vi "ZM-CI-handlePackage.vi"(8 "error in (no error)":errorcluster, 10 "package":refnum<class "ZM-PC-package.lvclass">, 11 "ZM-ROOT-root in":refnum<class "ZM-ROOT-root.lvclass">) -> (0 "error out":errorcluster, 3 "ZM-ROOT-root out":refnum<class "ZM-ROOT-root.lvclass">)   [LabVIEW 2020, in "ZM-ROOT-root.lvlib" / "ZM-ROOT-root.lvclass"]
doc: "The root's ZM-CI-handlePackage override: routes every package by destination. Communication: noted and forwarded to the communication manager while it runs. Root: an error package is shown on the panel, any other is noted. Unknown and Hardware: dropped with one line in the error log (not an error)."
uses:
  ZM-ROOT-root.lvclass
  common/ZM-PC-packages/ZM-PC-package/ZM-PC-package.lvclass
  ZM-ROOT-root.lvclass/ZM-ROOT-root.ctl
  common/ZM-CI-common_interfaces/ZM-CI-handlePackage Msg/ZM-CI-handlePackage Msg.lvclass
  <vilib>/ActorFramework/Message Enqueuer/Message Enqueuer.lvclass
  common/ZM-CU-common_utilities/ZM-CU-common_utilities.lvlib
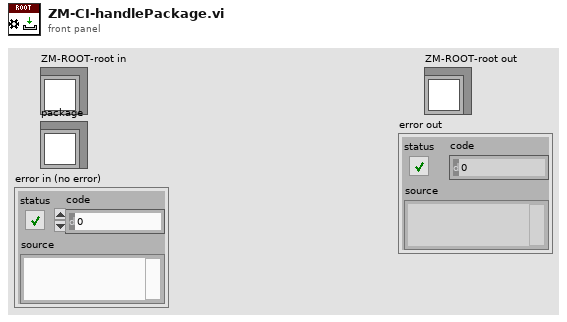
[diagram p1: front panel]
types:
  T1 = typedef "ZM-PC-packages.lvlib/ZM-PC-package.lvclass/ZM-PC-DESTINATION.ctl" = enum16{"Unknown", "Root", "Hardware", "Communication"}
  T2 = typedef "ZM-PC-packages.lvlib/ZM-PC-package.lvclass/ZM-PC-PACKAGE_TYPE.ctl" = enum16{"Undefined", "TestPackage", "ErrorPackage"}
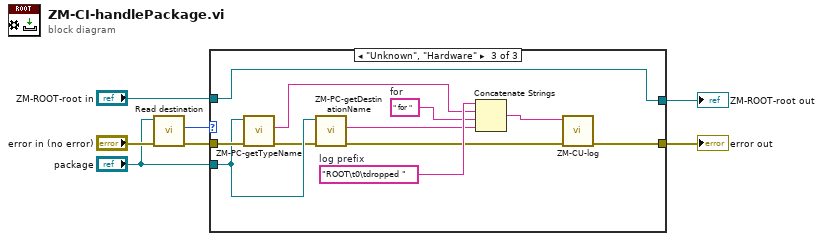
[diagram p0: block diagram]
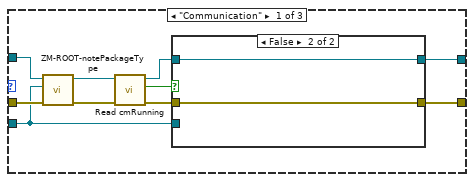
[diagram p2: hidden frame]
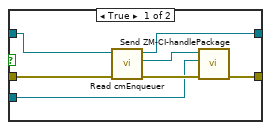
[diagram p3: hidden frame]
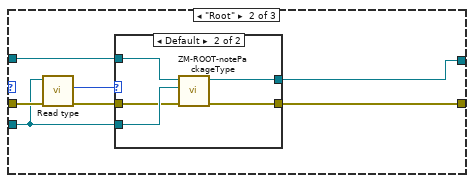
[diagram p4: hidden frame]
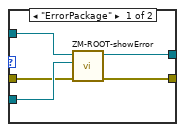
[diagram p5: hidden frame]
diagram:
  n1 = call "Read destination.vi"("error in (no error)"="error in (no error)", "ZM-PC-package in"="package") -> ("error out"=w4:errorcluster, "ZM-PC-DESTINATION"=w3:T1)  [unwired: 7 in, 1 out]
  n2 = case shown="\"Unknown\", \"Hardware\"" w3 {
    tunnel: "ZM-ROOT-root in" -> [w17 w32 w45]
    tunnel: "package" -> [w12 w31 w53]
    tunnel: w4 -> [w16 w33 w54]
    tunnel: [w9 w28 w45] -> w2
    tunnel: [w8 w27 w44] -> w1
    frame "Communication" {
      n3 = call "ZM-ROOT-notePackageType.vi"("error in (no error)"=w16, "package"=w12, "ZM-ROOT-root in"=w17) -> ("error out"=w15:errorcluster, "ZM-ROOT-root out"=w14:refnum<class "ZM-ROOT-root.lvclass">)  [unwired: 7 in]
      n4 = call "Read cmRunning.vi"("error in (no error)"=w15, "ZM-ROOT-root in"=w14) -> ("error out"=w11:errorcluster, "cmRunning"=w10:bool, "ZM-ROOT-root out"=w13:refnum<class "ZM-ROOT-root.lvclass">)  [unwired: 7 in]
      n5 = case shown="False" w10 {
        tunnel: w13 -> [w23 w26]
        tunnel: w12 -> [w20 _]
        tunnel: w11 -> [w24 w25]
        tunnel: [w19 w26] -> w9
        tunnel: [w18 w25] -> w8
        frame True {
          n6 = call "Read cmEnqueuer.vi"("error in (no error)"=w24, "ZM-ROOT-root in"=w23) -> ("error out"=w21:errorcluster, "Actor Framework:Message Enqueuer"=w22:refnum<class "Message Enqueuer.lvclass">, "ZM-ROOT-root out"=w19:refnum<class "ZM-ROOT-root.lvclass">)  [unwired: 7 in]
          n7 = call "Send ZM-CI-handlePackage.vi"("error in (no error)"=w21, "package"=w20, "Message Enqueuer"=w22) -> ("error out"=w18:errorcluster)  [unwired: 7 in, 1 out]
        }
        frame False {
        }
      }
    }
    frame "Root" {
      n8 = call "Read type.vi"("error in (no error)"=w33, "ZM-PC-package in"=w31) -> ("error out"=w30:errorcluster, "ZM-PC-PACKAGE_TYPE"=w29:T2)  [unwired: 7 in, 1 out]
      n9 = case shown="Default" w29 {
        tunnel: w32 -> [w38 w43]
        tunnel: w31 -> [w37 w42]
        tunnel: w30 -> [w36 w41]
        tunnel: [w35 w40] -> w28
        tunnel: [w34 w39] -> w27
        frame "ErrorPackage" {
          n10 = call "ZM-ROOT-showError.vi"("error in (no error)"=w36, "package"=w37, "ZM-ROOT-root in"=w38) -> ("error out"=w34:errorcluster, "ZM-ROOT-root out"=w35:refnum<class "ZM-ROOT-root.lvclass">)  [unwired: 7 in]
        }
        frame Default {
          n11 = call "ZM-ROOT-notePackageType.vi"("error in (no error)"=w41, "package"=w42, "ZM-ROOT-root in"=w43) -> ("error out"=w39:errorcluster, "ZM-ROOT-root out"=w40:refnum<class "ZM-ROOT-root.lvclass">)  [unwired: 7 in]
        }
      }
    }
    frame "Unknown", "Hardware" {
      w49 = " for "  # for
      w51 = "ROOT\t0\tdropped "  # log prefix
      n12 = call "ZM-PC-getTypeName.vi"("error in (no error)"=w54, "ZM-PC-package in"=w53) -> ("error out"=w52:errorcluster, "type_name"=w50:string)  [unwired: 7 in, 1 out]
      n13 = call "ZM-PC-getDestinationName.vi"("error in (no error)"=w52, "ZM-PC-package in"=w53) -> ("error out"=w46:errorcluster, "destination_name"=w48:string)  [unwired: 7 in, 1 out]
      n14 = Concatenate Strings(w51, w50, w49, w48) -> (w47:string)
      n15 = call "ZM-CU-log.vi"("error in"=w46, "message"=w47) -> ("error out"=w44:errorcluster)  [unwired: 9 in]
    }
  }
  "ZM-ROOT-root out" <- w2
  "error out" <- w1
